vi "Test Client Recovers After Timeout.vi"(8 "error in (no error)":errorcluster) -> (0 "error out":errorcluster)   [LabVIEW 2019, in "RemoteControl.ZMQ.Tests.lvclass"]
uses:
  RemoteControl.ZMQ.Tests.lvclass
  C:/Program Files/National Instruments/LabVIEW 2019/user.lib/LevyLab/RemoteControl/RemoteControl/RemoteControl.lvclass
  <userlib>/LevyLab/RemoteControl/RemoteControl/RemoteControl.lvclass/RemoteControl.ctl
  <vilib>/numeric/Random Number (Range) U64.vi
  <vilib>/numeric/sub_Random U32.vi
  <vilib>/addons/_JKI Toolkits/Caraya/classes/Assert/Assert True.vi
  <vilib>/addons/_JKI Toolkits/Caraya/classes/Assert/Assert Not Error.vi
  <userlib>/LevyLab/RemoteControl/RemoteControl/RemoteControl.lvclass
  <vilib>/addons/_JKI Toolkits/Caraya/classes/Assert/Assert.lvclass
  <vilib>/addons/_JKI Toolkits/Caraya/classes/Test/Test.lvclass
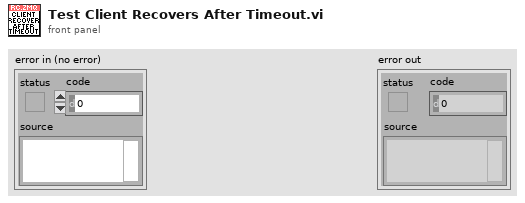
[diagram p1: front panel]
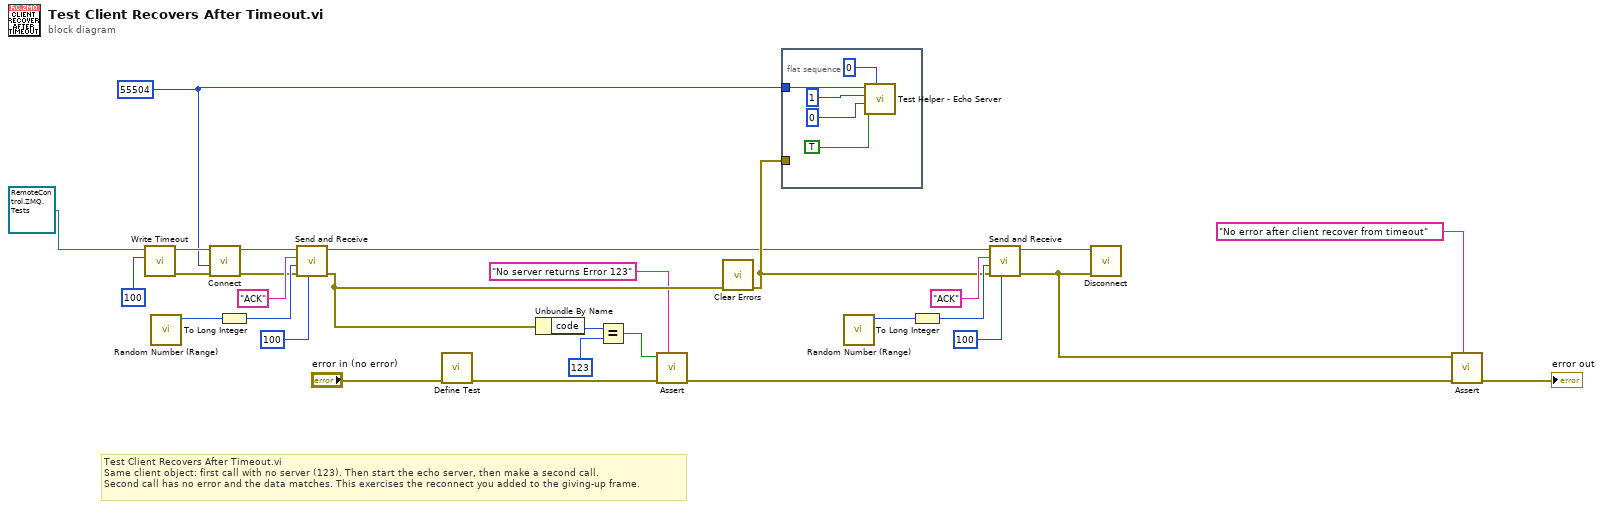
[diagram p0: block diagram]
diagram:
  w17 = u16 55504 ("Port")
  # "Test Client Recovers After Timeout.vi\nSame client object: first call with no server (123). Then start the echo server, then make a second call.\nSecond call has no error and the data matches. This exercises the reconnect you added to the giving-up frame."
  n1 = call <userlib>:"Write Timeout.vi"("timeout (ms) [500]"=100 ("timeout in ms (100)"), "RemoteControl in"=refnum<class "RemoteControl.ZMQ.Tests.lvclass"> refnum ("RemoteControl.ZMQ.lvlib:RemoteControl.ZMQ.Tests.lvclass")) -> ("error out"=w23:errorcluster, "RemoteControl out"=w22:refnum<class "RemoteControl.ZMQ.Tests.lvclass">)  [unwired: 8 in]
  n2 = call-poly <vilib>:"Random Number (Range).vi"() -> ("number"=w25:u64)  [unwired: 11 in]
  n3 = call <userlib>:"Connect.vi"("error in (no error)"=w23, "Port"=w17, "RemoteControl in"=w22) -> ("error out"=w16:errorcluster, "RemoteControl out"=w29:refnum<class "RemoteControl.ZMQ.Tests.lvclass">)  [unwired: 7 in]
  n4 = To Long Integer(number=w25) -> (32bit integer=w20:i32)
  n5 = call <userlib>:"Send and Receive.vi"("timeout (ms) [500]"=100, "error in (no error)"=w16, "Data"=w20, "Command"="ACK", "RemoteControl in"=w29) -> ("error out"=w28:errorcluster, "RemoteControl out"=w3:refnum<class "RemoteControl.ZMQ.Tests.lvclass">)  [unwired: 3 in, 2 out]
  n6 = call <vilib>:"Define Test.vi"("error in (no error)"="error in (no error)") -> ("error out"=w11:errorcluster)  [unwired: 9 in, 1 out]
  n7 = Unbundle By Name(w28) -> ("code"=w14:i32)
  n8 = Equal?(x=w14, y=123 ("error code (1)")) -> (x = y?=w12:bool)
  n9 = call-poly <vilib>:"Assert.vi"("Label"="No server returns Error 123", "error in (no error)"=w11, "True?"=w12) -> ("error out"=w5:errorcluster)  [unwired: 7 in, 1 out]
  n10 = call <vilib>:"Clear Errors.vi"("error in (no error)"=w28) -> ("error out"=w4:errorcluster)  [unwired: 5 in, 1 out]
  n11 = flat-sequence {
    tunnel: w17 -> [w31]
    tunnel: w4 -> [_]
    frame #0 {
      n12 = call "Test Helper - Echo Server.vi"("idle timout"=u32 0, "Answer?"=TRUE, "reply delay (ms)"=u32 0, "number of messages"=1, "port"=w31) -> ()  [unwired: 5 in, 2 out]
    }
  }
  n13 = call-poly <vilib>:"Random Number (Range).vi"() -> ("number"=w9:u64)  [unwired: 11 in]
  n14 = To Long Integer(number=w9) -> (32bit integer=w7:i32)
  n15 = call <userlib>:"Send and Receive.vi"("timeout (ms) [500]"=100, "error in (no error)"=w4, "Data"=w7, "Command"="ACK", "RemoteControl in"=w3) -> ("error out"=w1:errorcluster, "RemoteControl out"=w10:refnum<class "RemoteControl.ZMQ.Tests.lvclass">)  [unwired: 3 in, 2 out]
  n16 = call <userlib>:"Disconnect.vi"("error in (no error)"=w1, "RemoteControl in"=w10) -> ()  [unwired: 8 in, 2 out]
  n17 = call-poly <vilib>:"Assert.vi"("Label"="No error after client recover from timeout", "error in (no error)"=w5, "Not Error?"=w1) -> ("error out"=→"error out":errorcluster)  [unwired: 7 in, 1 out]
